vi "Read ActivationHandler.vi"(8 "error in (no error)":errorcluster, 11 "ToastService in":refnum<class "ToastService.lvclass">) -> (0 "error out":errorcluster, 2 "ActivationHandler":refnum<class "ActivationHandler.lvclass">, 3 "ToastService out":refnum<class "ToastService.lvclass">)   [LabVIEW 2026, in "ToastNotification.lvlib" / "ToastService.lvclass"]
doc: "Return the handler stored by ToastService.Initialize, including references created by its Initialize hook. The caller borrows these resources; ToastService.Close calls the handler Close hook. This accessor does not initialize a new handler or transfer resource ownership."
uses:
  ToastService.lvclass
  ActivationHandler/ActivationHandler.lvclass
  ToastService.lvclass/ToastService.ctl
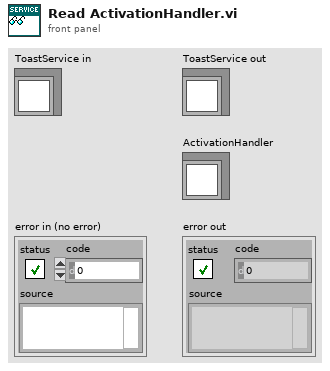
[diagram p1: front panel]
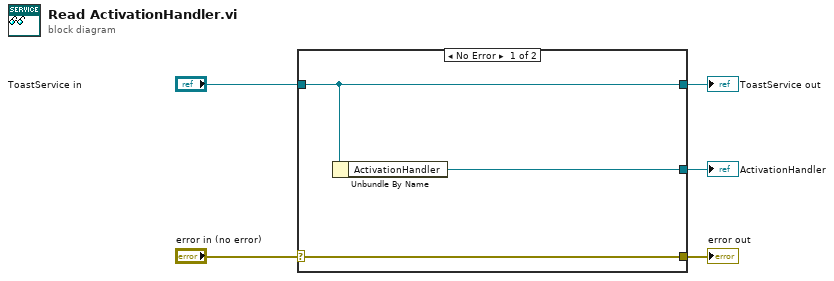
[diagram p0: block diagram]
diagram:
  n1 = case shown="No Error" "error in (no error)" {
    selector: "error in (no error)" -> [w8 w9]
    tunnel: [w8 w9] -> w4
    tunnel: [w7 w10] -> w2
    tunnel: "ToastService in" -> [w7 w10]
    tunnel: [w6 _] -> w1
    frame No Error {
      n2 = Unbundle By Name(w7) -> ("ActivationHandler"=w6:refnum<class "ActivationHandler.lvclass">)
    }
    frame Error {
    }
  }
  "error out" <- w4
  "ToastService out" <- w2
  "ActivationHandler" <- w1
